vi "CreateClass.vi"(0 "ClassWriterNative":refnum<class "ClassWriterNative.lvclass">, 1 "ProjectTreePosition(String or Project Item Ref)":variant, 2 "CreateClassData":T1, 5 "error in (no error)":errorcluster, 6 "KeepLvClassRefOpen(False)":bool, 7 "HeaderToApply (take from VIRef or /use 2D-8bit header, Ignored if not wired)":variant) -> (14 "ClassWriterNative":refnum<class "ClassWriterNative.lvclass">, 15 "LVClassLibraryRefnum":refnum<vi>, 16 "TemplateVersionUsed":string, 19 "error out":errorcluster)   [LabVIEW 2020, in "ClassWriterNative.lvclass"]
uses:
  <resource>/Framework/Providers/Open_GDS/ClassProviders/Provider_LvNativeClass/ClassWriterNative_class/ClassWriterNative.lvclass
  <resource>/Framework/Providers/Open_GDS/ClassProviders/Provider_BaseClassInterface/CreateClassData.ctl
  <resource>/Framework/Providers/Open_GDS/ClassProviders/Provider_LvNativeClass/LvNativeProviderName.ctl
  <resource>/Framework/Providers/Open_GDS/ClassProviders/Provider_LvNativeClass/Templates/LvNativeTemplateNames.ctl
  <vilib>/Utility/miscctls.llb/LVPositionTypeDef.ctl
  <resource>/Framework/Providers/Open_GDS/ClassProviders/Common/LvClass_class/GDSLvCLass_ClassSettingsType.ctl
  <resource>/Framework/Providers/Open_GDS/ClassProviders/Common/LvClass_class/GDSLvClass_PlugIn.ctl
  <resource>/Framework/Providers/Open_GDS/ClassProviders/Common/LvClass_class/GDSLvClass_PlugInTypes.ctl
  <resource>/Framework/Providers/Open_GDS/ClassProviders/Provider_LvNativeClass/ClassWriterNative_class/ClassWriterNative.lvclass/ClassWriterNative.ctl
  <resource>/Framework/Providers/Open_GDS/ClassProviders/Provider_BaseClassInterface/ClassWriter_class/ClassWriter.lvclass
  <vilib>/Utility/lvfile.llb/NI_FileType.lvlib
  <resource>/Framework/Providers/Open_GDS/ClassProviders/Common/InterfaceLibrary/InterfaceLibrary.lvlib
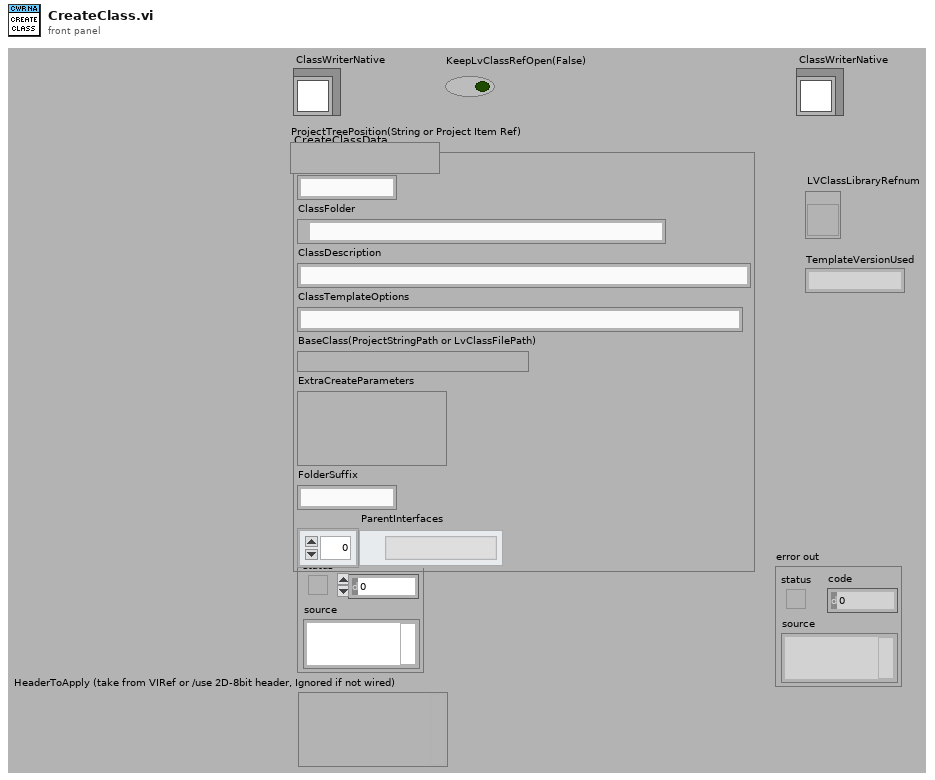
[diagram p1: front panel]
types:
  T1 = typedef "ClassWriter.lvclass/CreateClassData.ctl" = cluster{"ClassName":string, "ClassFolder":path, "ClassDescription":string, "ClassTemplateOptions":string, "BaseClass(ProjectStringPath or LvClassFilePath)":variant, "ExtraCreateParameters":variant, "FolderSuffix":string, "ParentInterfaces":path[]}
  T2 = cluster{"SubClass":bool, "ClassTemplateFiles":path[], "ClassName":string, "ClassFolder":path, "VIs":refnum<vi>[], "TemplateFolder":path, "ViSubDirs":string[], "TemplateName":string, "BaseClassFolder":path, "RootBaseClassFolder":path, "TemplateClass":refnum<vi>, "LvClassPath":path, "ClassRefnum":refnum<vi>, "ProjectRefnum":refnum<vi>, "LvClassFolderPath":path, "BaseClassName":string, "TemplateVersionUsed":string, "App":refnum<vi>}
  T3 = typedef "LvNativeProviderName.ctl" = enum16{"Endevo LabVIEW Native"}
  T4 = enum32{"invalid scope", "public", "private", "protected"}
  T5 = typedef "LVPositionTypeDef.ctl" = cluster{"Left":i32, "Top":i32}
  T6 = typedef "LvNativeTemplateNames.ctl" = enum16{"NativeBaseTemplate", "NativeSubTemplate", "NativeBaseTemplate_4x4x4", "NativeSubTemplate_4x4x4"}
  T7 = typedef "GDSLvCLass_ClassSettingsType.ctl" = cluster{"ClassProviderName":string, "ClassTemplateUsed":string, "ClassTemplateVersion":string, "ClassDescription":string, "PlugIns":T8[], "ConnectorPanePattern":string}
  T8 = typedef "GDSLvClass_PlugIn.ctl" = cluster{"Type":T9, "ID":string, "Version":string, "Path":path, "Name":string, "Data":variant}
  T9 = typedef "GDSLvClass_PlugInTypes.ctl" = enum16{"DesignPattern", "MethodTypes"}
  T10 = typedef "ClassWriter.lvclass/TemplateSettings.ctl" = cluster{"CommonClassTemplate":bool, "DynamicDispatch":enum8{"False", "True", "Mixed"}, "MustOverride":enum8{"False", "True", "Mixed"}, "MustCallParent":enum8{"False", "True", "Mixed"}, "OnlyNormalMethod":bool, "OnlyPublic":bool}
  T11 = cluster{"Major":u16, "Minor":u16, "Fix":u16, "Build":u16}
  T12 = typedef "Scripting_ConnectorPanePatternType.ctl" = u16
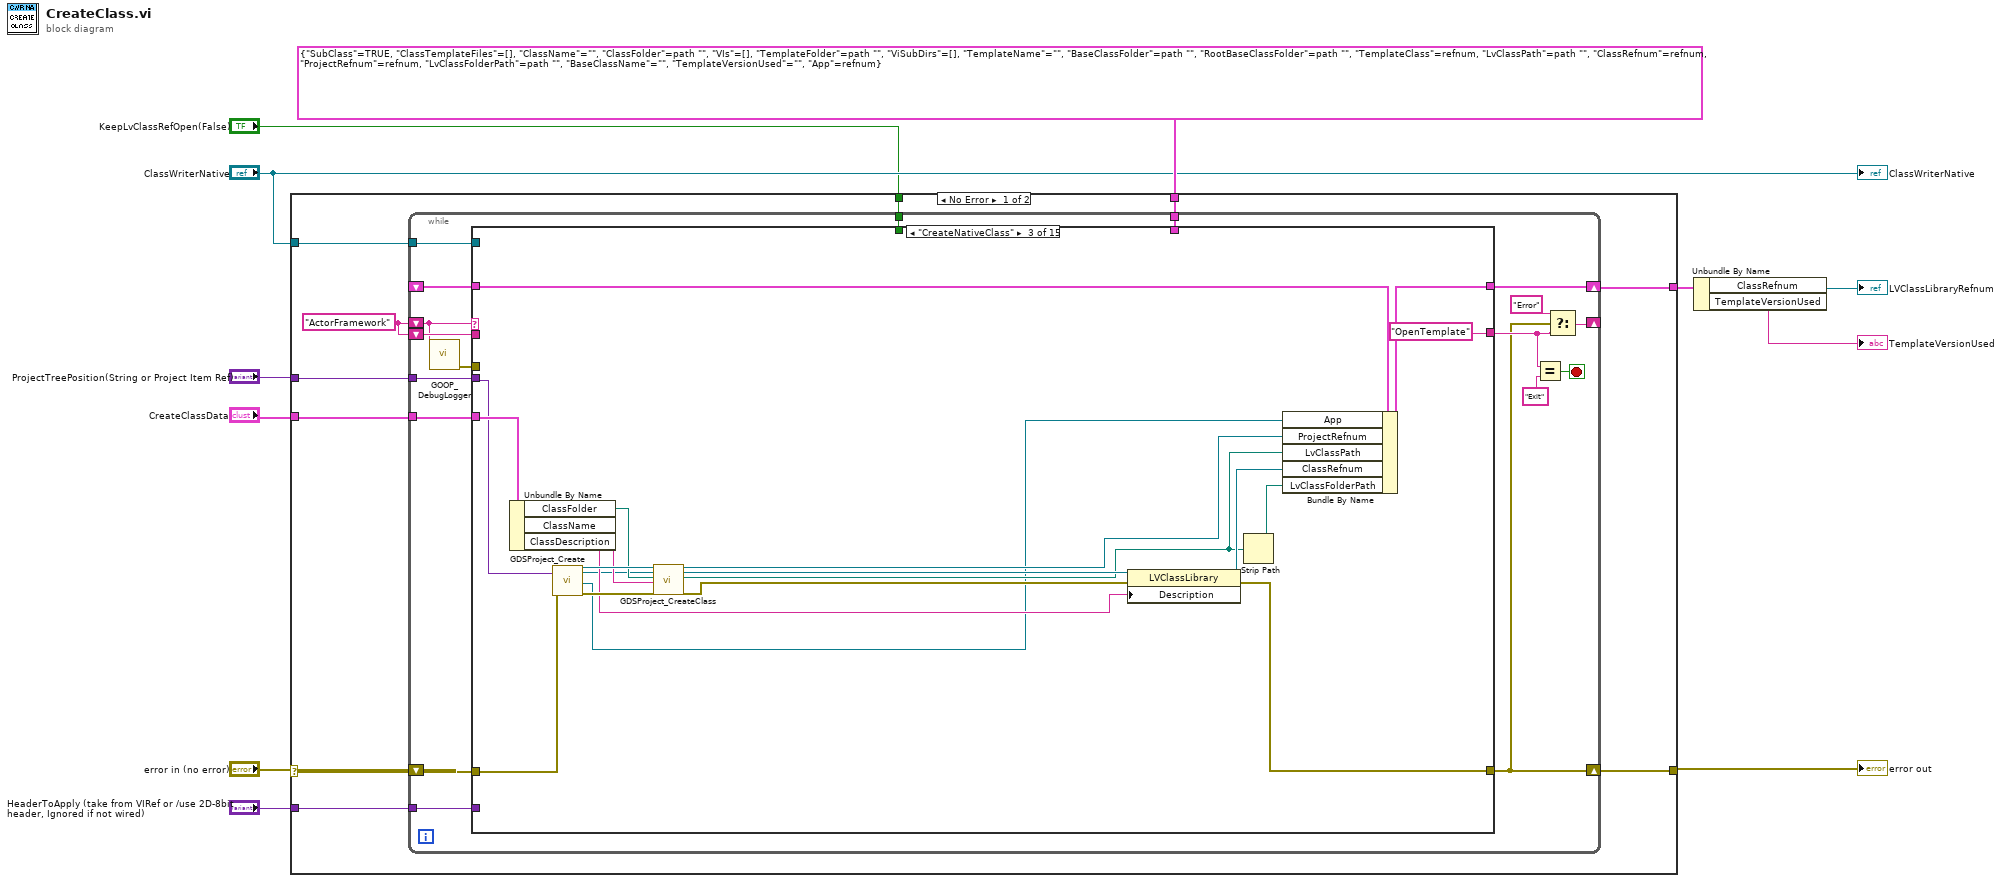
[diagram p0: block diagram]
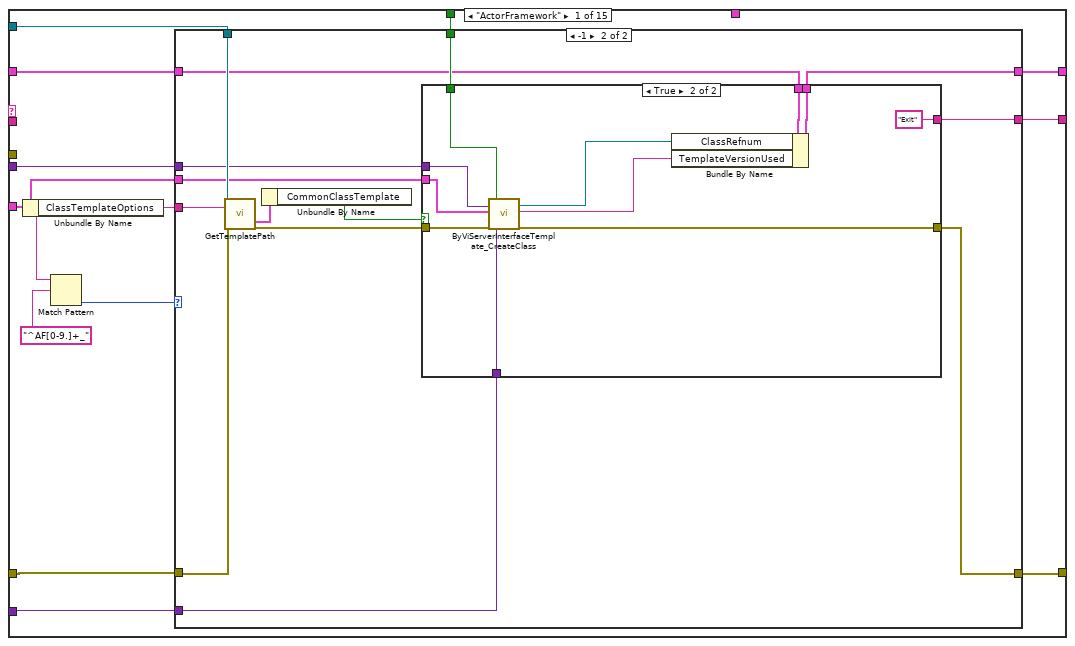
[diagram p2: hidden frame]
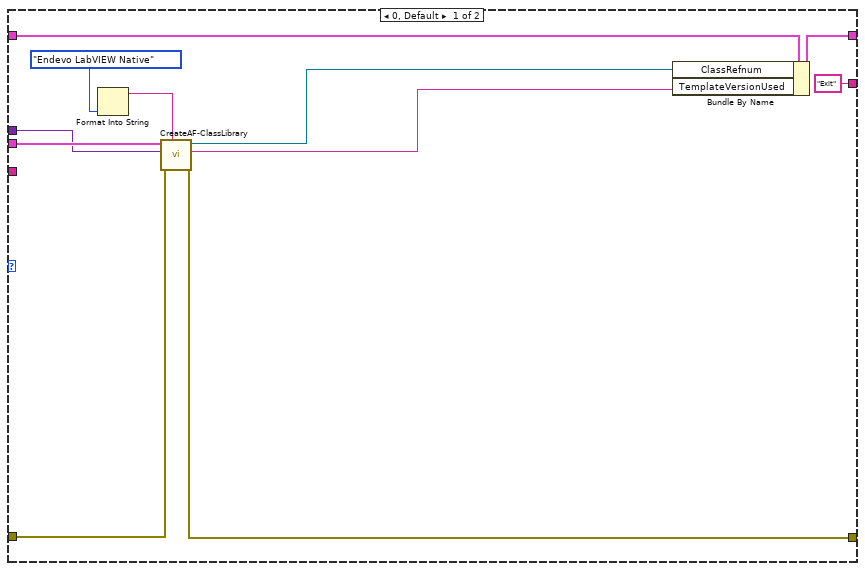
[diagram p3: hidden frame]
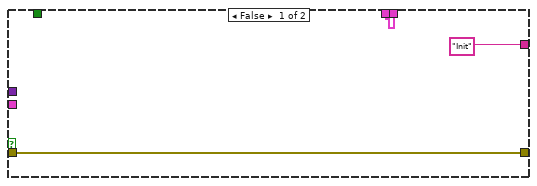
[diagram p4: hidden frame]
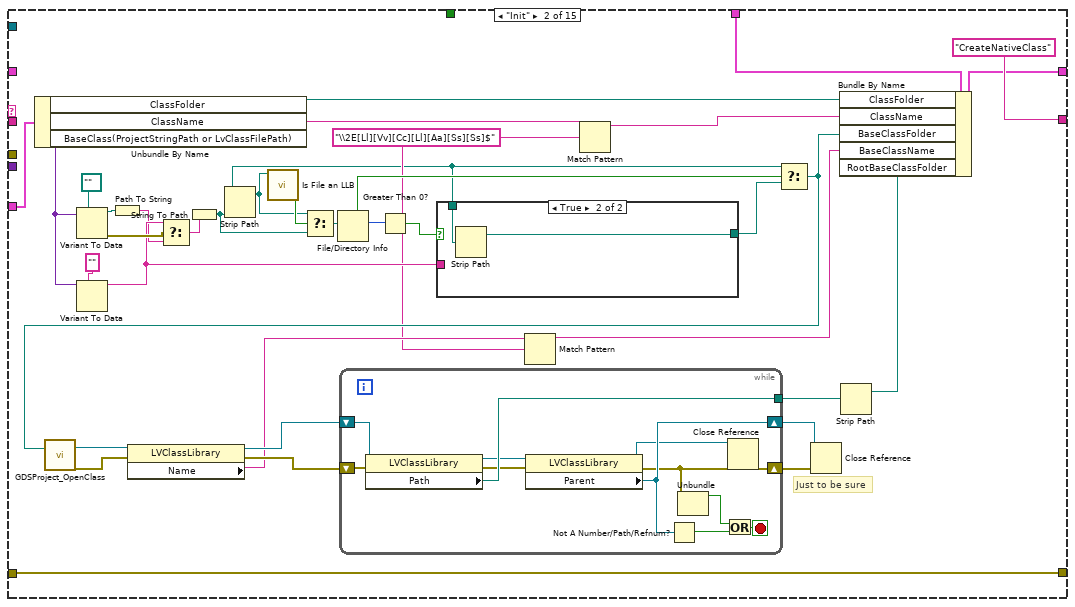
[diagram p5: hidden frame]
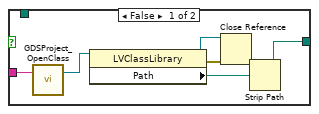
[diagram p6: hidden frame]
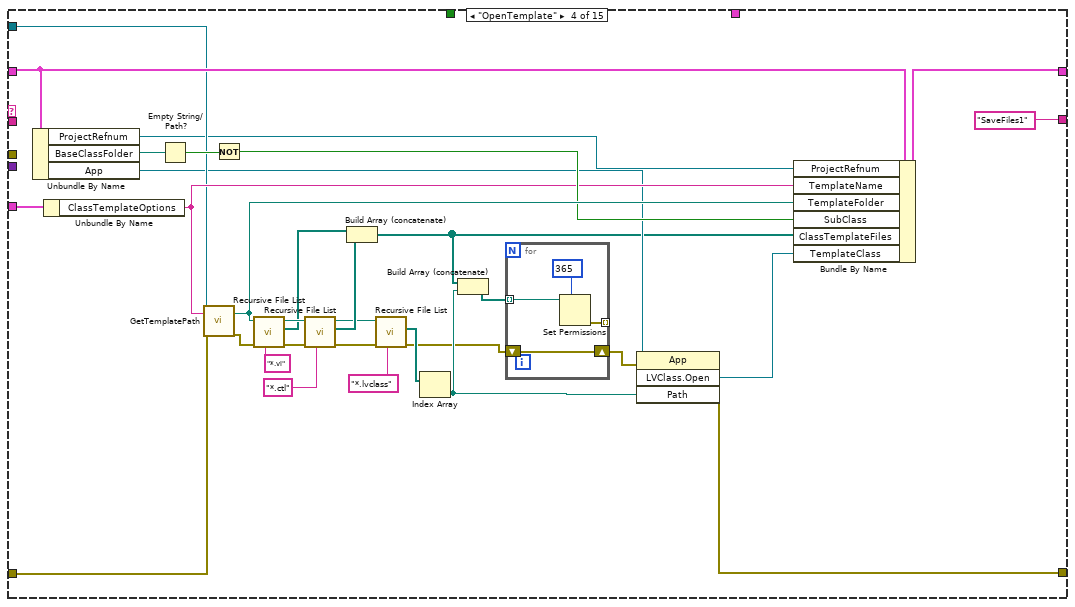
[diagram p7: hidden frame]
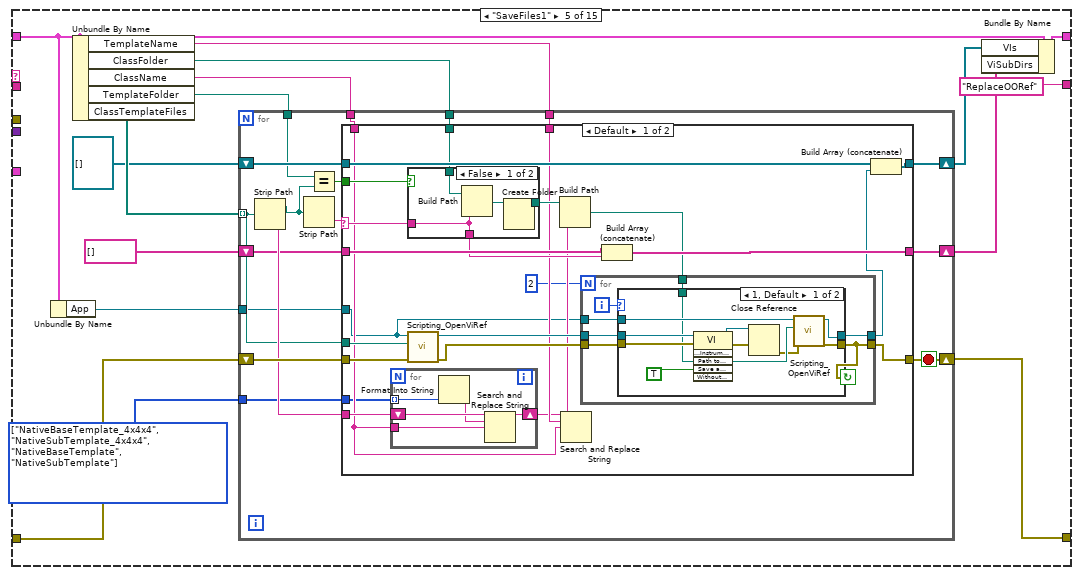
[diagram p8: hidden frame]
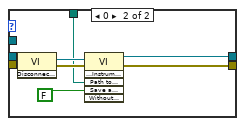
[diagram p9: hidden frame]
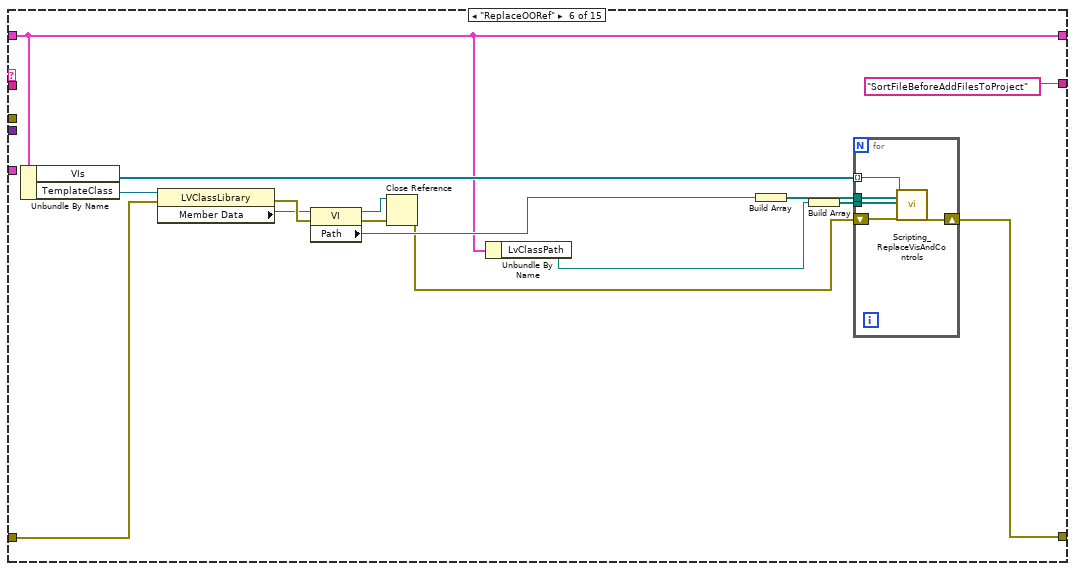
[diagram p12: hidden frame]
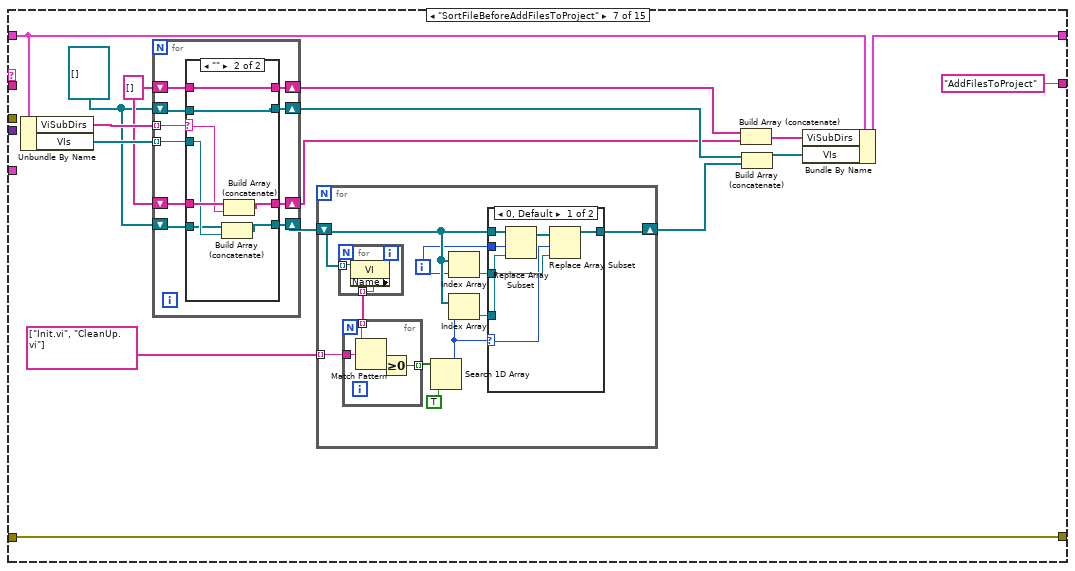
[diagram p13: hidden frame]
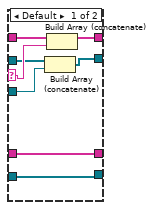
[diagram p15: hidden frame]
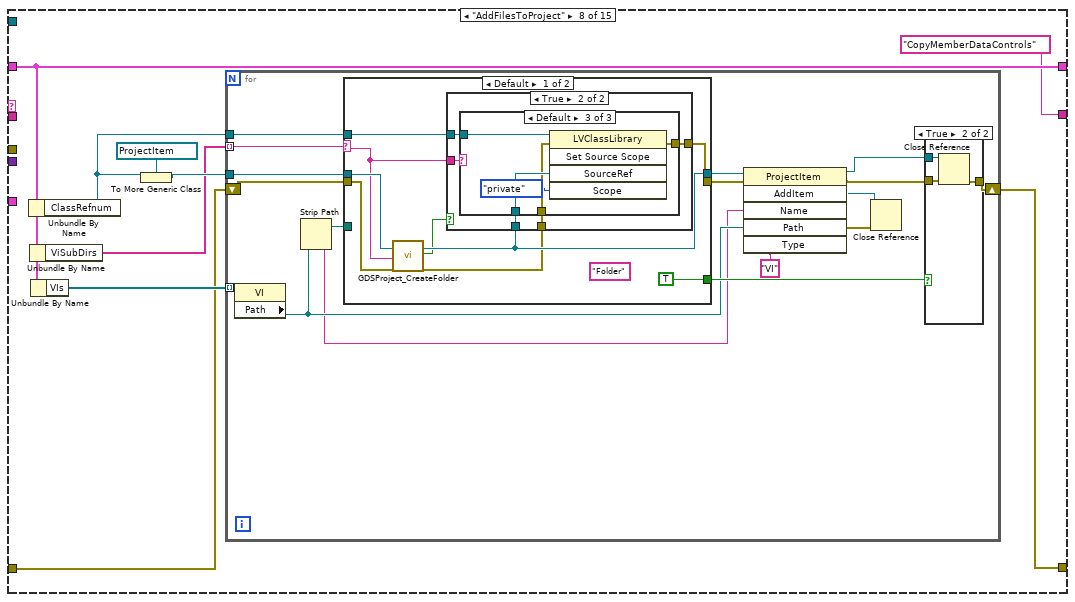
[diagram p16: hidden frame]
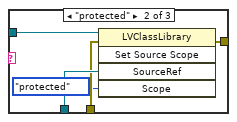
[diagram p20: hidden frame]
diagram:
  n1 = case shown="No Error" "error in (no error)" {
    selector: "error in (no error)" -> [w21 w687]
    tunnel: [w20 w687] -> w7
    tunnel: T2 {"SubClass"=TRUE, "ClassTemplateFiles"=[], "ClassName"="", "ClassFolder"=path "", "VIs"=[], "TemplateFolder"=path "", "ViSubDirs"=[], "TemplateName"="", "BaseClassFolder"=path "", "RootBaseClassFolder"=path "", "TemplateClass"=refnum, "LvClassPath"=path "", "ClassRefnum"=refnum, "ProjectRefnum"=refnum, "LvClassFolderPath"=path "", "BaseClassName"="", "TemplateVersionUsed"="", "App"=refnum} ("output cluster") -> [w19 _]
    tunnel: "ProjectTreePosition(String or Project Item Ref)" -> [w18 _]
    tunnel: "CreateClassData" -> [w17 _]
    tunnel: "ClassWriterNative" -> [w16 _]
    tunnel: "HeaderToApply (take from VIRef or /use 2D-8bit header, Ignored if not wired)" -> [w15 _]
    tunnel: "KeepLvClassRefOpen(False)" -> [w14 _]
    tunnel: [w13 _] -> w3
    frame No Error {
      w12 = "ActorFramework"
      n2 = while {
        shift-right: [w30] -> w20
        shift-left: w21 -> [w39]
        shift-right: [w34] -> _
        shift-left: w12 -> [w23]
        shift-right: [w37] -> w13
        shift-left: _ -> [w38]
        tunnel: w19 -> [w32]
        tunnel: w18 -> [w29]
        tunnel: w17 -> [w28]
        tunnel: w16 -> [w27]
        shift-left: w12 -> [w26]
        tunnel: w15 -> [w25]
        tunnel: w14 -> [w24]
        stop <- w35 stop-if-true
        n3 = call <resource>:"GOOP_DebugLogger.vi"("State"=w23) -> ("error out"=w22:errorcluster)  [unwired: 8 in, 2 out]
        n4 = case shown="\"CreateNativeClass\"" w23 {
          selector: w23 -> [_ _ _ _ _ _ _ _ _ _ _ _ _ _ w662]
          tunnel: w38 -> [w50 _ w154 w183 w206 w299 w331 w386 w491 w506 w525 w546 w560 w637 w659]
          tunnel: [w47 w124 w153 w197 w212 w299 w330 w386 w491 w506 w525 w546 w559 w637 w659] -> w37
          tunnel: w39 -> [w48 w127 w156 w177 w203 w305 w329 w384 w451 w497 w518 w544 w566 w615 w668]
          tunnel: [w45 w127 w152 w172 w202 w310 w329 w391 w441 w494 w529 w538 w583 w616 w661] -> w30
          tunnel: [w46 "CreateNativeClass" "OpenTemplate" "SaveFiles1" "ReplaceOORef" "SortFileBeforeAddFilesToProject" "AddFilesToProject" "CopyMemberDataControls" "UpdateIcons" w508 "AddFolders" "SetClassProperties" "FixAttribute" "CloseRefs" "Exit"] -> w31
          tunnel: w32 -> [_ w112 _ _ _ _ _ _ _ _ _ _ _ _ _]
          tunnel: w29 -> [w44 _ w155 _ _ _ _ _ _ _ _ _ _ _ _]
          tunnel: w28 -> [w49 w111 w157 w179 _ _ _ _ _ _ _ _ w580 _ _]
          tunnel: w27 -> [w42 _ _ w180 _ _ _ _ _ w493 w520 _ _ _ _]
          tunnel: w26 -> [_ _ _ _ _ _ _ _ _ _ _ _ _ _ w660]
          tunnel: w25 -> [w40 _ _ _ _ _ _ _ _ w502 _ _ _ _ _]
          tunnel: w24 -> [w41 _ _ _ _ _ _ _ _ _ _ _ _ _ w657]
          tunnel: w22 -> [_ _ _ _ _ _ _ _ _ _ _ _ _ _ _]
          frame "ActorFramework" {
            n5 = Unbundle By Name(w49) -> ("ClassTemplateOptions"=w43:string)
            n6 = Match Pattern(string=w43, regular expression="^AF[0-9.]+_") -> (offset past match=w52:i32)  [unwired: 1 in, 3 out]
            n7 = case shown="-1" w52 {
              tunnel: w50 -> [w63 w67]
              tunnel: [w62 w66] -> w47
              tunnel: ["Exit" w74] -> w46
              tunnel: w49 -> [w60 w69]
              tunnel: w48 -> [w59 w75]
              tunnel: [w58 w72] -> w45
              tunnel: w44 -> [w53 w70]
              tunnel: w43 -> [_ w77]
              tunnel: w42 -> [_ w76]
              tunnel: w41 -> [_ w71]
              tunnel: w40 -> [_ w68]
              frame 0, Default {
                n8 = Format Into String(LvNativeProviderName."Endevo LabVIEW Native" ("ProviderName")) -> (resulting string=w57:string)  [unwired: 3 in, 1 out]
                n9 = call <resource>:"CreateAF-ClassLibrary.vi"("Providername"=w57, "error in (no error)"=w59, "ProjectTreePosition(String or Project Item Ref)"=w53, "CreateClassData"=w60) -> ("error out"=w58:errorcluster, "TemplateVersionUsed"=w55:string, "LVClassLibraryRefnum"=w56:refnum<vi>)  [unwired: 5 in]
                n10 = Bundle By Name(cluster=w63, "ClassRefnum"=w56, "TemplateVersionUsed"=w55) -> (w62:T2)
              }
              frame -1 {
                n11 = call-dynamic "GetTemplatePath.vi"("reference in"=w76, "ClassTemplateSubDirectory"=w77, "error in (no error)"=w75) -> ("TemplateSettings"=w65:T10, "error out"=w73:errorcluster)  [unwired: 12 in, 3 out]
                n12 = Unbundle By Name(w65) -> ("CommonClassTemplate"=w64:bool)
                n13 = case shown="True" w64 {
                  tunnel: ["Init" "Exit"] -> w74
                  tunnel: w73 -> [w79 w90]
                  tunnel: [w79 w89] -> w72
                  tunnel: w71 -> [_ w88]
                  tunnel: w70 -> [_ w87]
                  tunnel: w69 -> [_ w86]
                  tunnel: w68 -> [_ w85]
                  tunnel: w67 -> [w78 w84]
                  tunnel: [w78 w83] -> w66
                  frame False {
                  }
                  frame True {
                    n14 = call <resource>:"ByViServerInterfaceTemplate_CreateClass.vi"("ProjectTreePosition(String or Project Item Ref)"=w87, "CreateClassData"=w86, "error in (no error)"=w90, "KeepLvClassRefOpen(False)"=w88, "HeaderToApply (take from VIRef or /use 2D-8bit header, Ignored if not wired)"=w85) -> ("LVClassLibraryRefnum"=w82:refnum<vi>, "TemplateVersionUsed"=w81:string, "error out"=w89:errorcluster)  [unwired: 12 in]
                    n15 = Bundle By Name(cluster=w84, "ClassRefnum"=w82, "TemplateVersionUsed"=w81) -> (w83:T2)
                  }
                }
              }
            }
          }
          frame "Init" {
            w97 = "\\2E[Ll][Vv][Cc][Ll][Aa][Ss][Ss]$" ("regular expression")
            # "Just to be sure"
            n16 = Unbundle By Name(w111) -> ("ClassFolder"=w110:path, "ClassName"=w109:string, "BaseClass(ProjectStringPath or LvClassFilePath)"=w108:variant)
            n17 = Variant To Data(type=path "" ("path"), Variant=w108) -> (data=w114:path, error out=w118:errorcluster)  [unwired: 1 in]
            n18 = Variant To Data(type="" ("regular expression"), Variant=w108) -> (data=w115:string)  [unwired: 1 in, 1 out]
            n19 = Path To String(path=w114) -> (string=w113:string)
            n20 = Select(t=w115, s=w118, f=w113) -> (s? t:f=w117:string)
            n21 = String To Path(string=w117) -> (path=w93:path)
            n22 = Strip Path(path=w93) -> (stripped path=w94:path)  [unwired: 1 out]
            n23 = call <vilib>:"Is File an LLB.vi"("path"=w94) -> ("Is LLB?"=w95:bool)  [unwired: 9 in, 1 out]
            n24 = Select(t=w94, s=w95, f=w93) -> (s? t:f=w92:path)
            n25 = File/Directory Info(path=w92) -> (directory=w122:bool, size=w121:i64)  [unwired: 1 in, 5 out]
            n26 = Greater Than 0?(x=w121) -> (x > 0?=w119:bool)
            n27 = case shown="True" w119 {
              tunnel: w93 -> [_ w146]
              tunnel: [w143 w145] -> w120
              tunnel: w115 -> [w144 _]
              frame False {
                n28 = call <resource>:"GDSProject_OpenClass.vi"("ClassPath(FilePath/ProjectTreePath/LvCLassRef)"=w144) -> ("LVClass.Open"=w141:refnum<vi>)  [unwired: 16 in, 2 out]
                n29 = property class="LVClassLibrary"(reference=w141) -> (reference out=w139:refnum<vi>, error out=w140:errorcluster, "Path"=w142:path)  [unwired: 1 in]
                n30 = Close Reference(reference=w139, error in (no error)=w140) -> ()  [unwired: 1 out]
                n31 = Strip Path(path=w142) -> (stripped path=w143:path)  [unwired: 1 out]
              }
              frame True {
                n32 = Strip Path(path=w146) -> (stripped path=w145:path)  [unwired: 1 out]
              }
            }
            n33 = Match Pattern(string=w109, regular expression=w97) -> (before substring=w125:string)  [unwired: 1 in, 3 out]
            n34 = Select(t=w93, s=w122, f=w120) -> (s? t:f=w107:path)
            n35 = call <resource>:"GDSProject_OpenClass.vi"("ClassPath(FilePath/ProjectTreePath/LvCLassRef)"=w107) -> ("LVClass.Open"=w100:refnum<vi>, "error out"=w102:errorcluster)  [unwired: 16 in, 1 out]
            n36 = property class="LVClassLibrary"(reference=w100, error in=w102) -> (reference out=w99:refnum<vi>, error out=w101:errorcluster, "Name"=w98:string)
            n37 = while {
              shift-right: [w135] -> w106
              shift-left: w101 -> [w130]
              shift-right: [w136] -> w105
              shift-left: w99 -> [w138]
              tunnel: [w137] -> w104
              stop <- w132 stop-if-true
              n38 = property class="LVClassLibrary"(reference=w138, error in=w130) -> (reference out=w128:refnum<vi>, error out=w129:errorcluster, "Path"=w137:path)
              n39 = property class="LVClassLibrary"(reference=w128, error in=w129) -> (reference out=w131:refnum<vi>, error out=w135:errorcluster, "Parent"=w136:refnum<vi>)
              n40 = Not A Number/Path/Refnum?(number/path/refnum=w136) -> (NaN/Path/Refnum?=w133:bool)
              n41 = Unbundle(w135) -> ("status"=w134:bool)  [unwired: 2 out]
              n42 = Or(x=w134, y=w133) -> (x .or. y?=w132:bool)
              n43 = Close Reference(reference=w131) -> ()  [unwired: 1 in, 1 out]
            }
            n44 = Match Pattern(string=w98, regular expression=w97) -> (before substring=w96:string)  [unwired: 1 in, 3 out]
            n45 = Close Reference(reference=w105, error in (no error)=w106) -> ()  [unwired: 1 out]
            n46 = Strip Path(path=w104) -> (stripped path=w103:path)  [unwired: 1 out]
            n47 = Bundle By Name(cluster=w112, "ClassFolder"=w110, "ClassName"=w125, "BaseClassFolder"=w107, "BaseClassName"=w96, "RootBaseClassFolder"=w103) -> (w124:T2)
          }
          frame "CreateNativeClass" {
            n48 = Unbundle By Name(w157) -> ("ClassFolder"=w161:path, "ClassName"=w162:string, "ClassDescription"=w158:string)
            n49 = call <resource>:"GDSProject_Create.vi"("ProjectTreePosition(String or Project Item Ref)"=w155, "error in (no error)"=w156) -> ("Project Refnum"=w165:refnum<vi>, "Project Item"=w151:refnum<vi>, "App"=w147:refnum<vi>, "error out"=w164:errorcluster)  [unwired: 13 in, 1 out]
            n50 = call <resource>:"GDSProject_CreateClass.vi"("Project Refnum In"=w165, "Project Item To Create Class Below(Use MyComputer if not wired)"=w151, "ClassFolder"=w161, "ClassName"=w162, "error in (no error)"=w164) -> ("Project Refnum Out"=w149:refnum<vi>, "Class Refnum Out"=w160:refnum<vi>, "ClassPathOut"=w150:path, "error out"=w148:errorcluster)  [unwired: 11 in]
            n51 = property class="LVClassLibrary"(reference=w160, error in=w148, "Description"=w158) -> (reference out=w159:refnum<vi>, error out=w152:errorcluster)
            n52 = Strip Path(path=w150) -> (stripped path=w163:path)  [unwired: 1 out]
            n53 = Bundle By Name(cluster=w154, "App"=w147, "ProjectRefnum"=w149, "LvClassPath"=w150, "ClassRefnum"=w159, "LvClassFolderPath"=w163) -> (w153:T2)
          }
          frame "OpenTemplate" {
            n54 = Unbundle By Name(w183) -> ("ProjectRefnum"=w174:refnum<vi>, "BaseClassFolder"=w185:path, "App"=w173:refnum<vi>)
            n55 = Unbundle By Name(w179) -> ("ClassTemplateOptions"=w181:string)
            n56 = Empty String/Path?(string/path=w185) -> (empty?=w184:bool)
            n57 = call-dynamic "GetTemplatePath.vi"("reference in"=w180, "ClassTemplateSubDirectory"=w181, "error in (no error)"=w177) -> ("FolderPathOut"=w186:path, "error out"=w176:errorcluster)  [unwired: 12 in, 3 out]
            n58 = Not(x=w184) -> (.not. x?=w182:bool)
            n59 = call <vilib>:"Recursive File List.vi"("pattern"="*.vi", "error in (no error)"=w176, "Folder Path"=w186) -> ("error out"=w191:errorcluster, "All Files in Dir"=w193:path[], "dup Folder Path"=w195:path)  [unwired: 4 in, 2 out]
            n60 = call <vilib>:"Recursive File List.vi"("pattern"="*.ctl", "error in (no error)"=w191, "Folder Path"=w195) -> ("error out"=w190:errorcluster, "All Files in Dir"=w192:path[], "dup Folder Path"=w189:path)  [unwired: 4 in, 2 out]
            n61 = Build Array (concatenate)(w193, w192) -> (w171:path[])
            n62 = call <vilib>:"Recursive File List.vi"("pattern"="*.lvclass", "error in (no error)"=w190, "Folder Path"=w189) -> ("error out"=w169:errorcluster, "All Files in Dir"=w187:path[])  [unwired: 4 in, 3 out]
            n63 = Index Array(array=w187) -> (element=w170:path)  [unwired: 1 in]
            n64 = Build Array (concatenate)(w171, w170) -> (w167:path[])
            n65 = for {
              tunnel: w167 -> [w200] mode=indexing
              shift-right: [w201] -> w168
              shift-left: w169 -> [w201]
              tunnel: [w198] -> _ mode=indexing
              n66 = Set Permissions(7:i16 365 ("permissions"), 11:w200) -> (0:w198:errorcluster)  [unwired: 3 in, 1 out]
            }
            n67 = invoke class="App" method="LVClass.Open"(reference=w173, error in=w168, "Path"=w170) -> (error out=w172:errorcluster, "LVClass.Open"=w175:refnum<vi>)  [unwired: 1 in, 2 out]
            n68 = Bundle By Name(cluster=w183, "ProjectRefnum"=w174, "TemplateName"=w181, "TemplateFolder"=w186, "SubClass"=w182, "ClassTemplateFiles"=w171, "TemplateClass"=w175) -> (w197:T2)
          }
          frame "SaveFiles1" {
            w205 = T6[] [enum."NativeBaseTemplate_4x4x4", enum."NativeSubTemplate_4x4x4", enum."NativeBaseTemplate", enum."NativeSubTemplate"] items=["NativeBaseTemplate", "NativeSubTemplate", "NativeBaseTemplate_4x4x4", "NativeSubTemplate_4x4x4"]
            n69 = Unbundle By Name(w206) -> ("App"=w204:refnum<vi>)
            n70 = Unbundle By Name(w206) -> ("TemplateName"=w207:string, "ClassFolder"=w216:path, "ClassName"=w215:string, "TemplateFolder"=w210:path, "ClassTemplateFiles"=w217:path[])
            n71 = for {
              tunnel: w217 -> [w223] mode=indexing
              shift-right: [w228] -> w213
              shift-left: refnum<vi>[] [] -> [w229]
              shift-right: [w218] -> w202
              shift-left: w203 -> [w233]
              tunnel: w216 -> [w232]
              tunnel: w215 -> [w230]
              tunnel: w210 -> [w225]
              shift-right: [w224] -> w208
              shift-left: string[] [] -> [w222]
              tunnel: w204 -> [w221]
              tunnel: w207 -> [w220]
              tunnel: w205 -> [w219]
              stop <- w218 stop-if-true
              n72 = Strip Path(path=w223) -> (stripped path=w227:path, name=w231:string)
              n73 = Strip Path(path=w227) -> (name=w234:string)  [unwired: 1 out]
              n74 = Equal?(x=w225, y=w227) -> (x = y?=w226:bool)
              n75 = case shown="Default" w234 {
                selector: w234 -> [w252 _]
                tunnel: w223 -> [w258 _]
                tunnel: w233 -> [w257 w295]
                tunnel: [w244 w295] -> w218
                tunnel: w232 -> [w253 _]
                tunnel: w231 -> [w256 _]
                tunnel: w230 -> [w239 _]
                tunnel: w229 -> [w255 w296]
                tunnel: [w254 w296] -> w228
                tunnel: w226 -> [w250 _]
                tunnel: [w248 w294] -> w224
                tunnel: w222 -> [w249 w294]
                tunnel: w221 -> [w236 _]
                tunnel: w220 -> [w240 _]
                tunnel: w219 -> [w237 _]
                frame Default {
                  n76 = for {
                    tunnel: w239 -> [w286]
                    shift-right: [w288] -> w238
                    shift-left: w256 -> [w287]
                    tunnel: w237 -> [w285] mode=indexing
                    n77 = Format Into String(w285) -> (resulting string=w284:string)  [unwired: 3 in, 1 out]
                    n78 = Search and Replace String(input string=w287, search string=w284, replace string=w286) -> (result string=w288:string)  [unwired: 5 in, 3 out]
                  }
                  n79 = case shown="False" w250 {
                    tunnel: w253 -> [w292 w293]
                    tunnel: w252 -> [w289 _]
                    tunnel: [w290 w293] -> w251
                    tunnel: [w289 _] -> w247
                    frame False {
                      n80 = Build Path(base path=w292, name or relative path=w289) -> (appended path=w291:path)
                      n81 = Create Folder(path (use dialog)=w291) -> (created path=w290:path)  [unwired: 2 in, 2 out]
                    }
                    frame True {
                    }
                  }
                  n82 = call <resource>:"Scripting_OpenViRef.vi"("error in"=w257, "ViPath/ViName/Viref"=w258, "AppRef"=w236) -> ("error out"=w246:errorcluster, "vi reference"=w245:refnum<vi>)  [unwired: 6 in, 1 out]
                  n83 = Search and Replace String(input string=w238, search string=w240, replace string=w239) -> (result string=w241:string)  [unwired: 5 in, 3 out]
                  n84 = Build Path(base path=w251, name or relative path=w241) -> (appended path=w242:path)
                  n85 = for {
                    N: 2 -> [_]
                    tunnel: w242 -> [w262]
                    tunnel: w236 -> [w261]
                    tunnel: w246 -> [w265]
                    tunnel: [w259] -> w244
                    tunnel: w245 -> [w264]
                    tunnel: [w263] -> w243
                    i -> [w260]
                    stop <- w259 continue-if-true
                    n86 = case shown="1, Default" w260 {
                      tunnel: w265 -> [w274 w283]
                      tunnel: w264 -> [w275 w282]
                      tunnel: [w270 w279] -> w259
                      tunnel: [w269 w278] -> w263
                      tunnel: w262 -> [w271 w277]
                      tunnel: w261 -> [w272 _]
                      frame 1, Default {
                        n87 = invoke class="VI" method="Save.Instrument"(reference=w275, error in=w274, "Path to saved file"=w271, "Save a Copy"=TRUE) -> (reference out=w267:refnum<vi>, error out=w268:errorcluster)  [unwired: 2 in, 4 out]
                        n88 = Close Reference(reference=w267, error in (no error)=w268) -> (error out=w266:errorcluster)
                        n89 = call <resource>:"Scripting_OpenViRef.vi"("error in"=w266, "ViPath/ViName/Viref"=w271, "AppRef"=w272) -> ("error out"=w270:errorcluster, "vi reference"=w269:refnum<vi>)  [unwired: 6 in, 1 out]
                      }
                      frame 0 {
                        n90 = invoke class="VI" method="DisconnectFromLibrary"(reference=w282, error in=w283) -> (reference out=w281:refnum<vi>, error out=w280:errorcluster)  [unwired: 1 in, 1 out]
                        n91 = invoke class="VI" method="Save.Instrument"(reference=w281, error in=w280, "Path to saved file"=w277, "Save a Copy"=FALSE) -> (reference out=w278:refnum<vi>, error out=w279:errorcluster)  [unwired: 2 in, 4 out]
                      }
                    }
                  }
                  n92 = Build Array (concatenate)(w249, w247) -> (w248:string[])
                  n93 = Build Array (concatenate)(w255, w243) -> (w254:refnum<vi>[])
                }
                frame "methods" {
                }
              }
            }
            n94 = Bundle By Name(cluster=w206, "VIs"=w213, "ViSubDirs"=w208) -> (w212:T2)
          }
          frame "ReplaceOORef" {
            n95 = Unbundle By Name(w299) -> ("VIs"=w311:refnum<vi>[], "TemplateClass"=w306:refnum<vi>)
            n96 = property class="LVClassLibrary"(reference=w306, error in=w305) -> (error out=w308:errorcluster, "Member Data"=w307:refnum<vi>)  [unwired: 1 out]
            n97 = property class="VI"(reference=w307, error in=w308) -> (reference out=w300:refnum<vi>, error out=w301:errorcluster, "Path"=w304:path)
            n98 = Close Reference(reference=w300, error in (no error)=w301) -> (error out=w297:errorcluster)
            n99 = Unbundle By Name(w299) -> ("LvClassPath"=w298:path)
            n100 = Build Array(w304) -> (w303:path[])
            n101 = Build Array(w298) -> (w302:path[])
            n102 = for {
              tunnel: w311 -> [w314] mode=indexing
              shift-right: [w315] -> w310
              shift-left: w297 -> [w316]
              tunnel: w302 -> [w313]
              tunnel: w303 -> [w312]
              n103 = call <resource>:"Scripting_ReplaceVisAndControls.vi"("ViRef"=w314, "OldVIsAndControls"=w312, "NewVIsAndControls"=w313, "error in (no error)"=w316) -> ("error out"=w315:errorcluster)  [unwired: 14 in, 1 out]
            }
          }
          frame "SortFileBeforeAddFilesToProject" {
            w321 = refnum<vi>[] []
            w322 = string[] []
            n104 = Unbundle By Name(w331) -> ("ViSubDirs"=w328:string[], "VIs"=w327:refnum<vi>[])
            n105 = for {
              tunnel: w328 -> [w366] mode=indexing
              tunnel: w327 -> [w361] mode=indexing
              shift-right: [w364] -> w326
              shift-left: w322 -> [w365]
              shift-right: [w362] -> w323
              shift-left: w321 -> [w363]
              shift-right: [w358] -> w320
              shift-left: w322 -> [w357]
              shift-right: [w360] -> w319
              shift-left: w321 -> [w359]
              n106 = case shown="\"\"" w366 {
                selector: w366 -> [w372 w378]
                tunnel: w365 -> [w374 w382]
                tunnel: [w373 w382] -> w364
                tunnel: w363 -> [w371 w381]
                tunnel: [w370 w381] -> w362
                tunnel: w361 -> [w369 w377]
                tunnel: w357 -> [w368 w380]
                tunnel: [w368 w379] -> w358
                tunnel: w359 -> [w367 w376]
                tunnel: [w367 w375] -> w360
                frame Default {
                  n107 = Build Array (concatenate)(w371, w369) -> (w370:refnum<vi>[])
                  n108 = Build Array (concatenate)(w374, w372) -> (w373:string[])
                }
                frame "" {
                  n109 = Build Array (concatenate)(w376, w377) -> (w375:refnum<vi>[])
                  n110 = Build Array (concatenate)(w380, w378) -> (w379:string[])
                }
              }
            }
            n111 = for {
              shift-right: [w338] -> w317
              shift-left: w319 -> [w342]
              tunnel: string[] ["Init.vi", "CleanUp.vi"] -> [w336] mode=indexing
              i -> [w341]
              n112 = for {
                tunnel: w342 -> [w356] mode=indexing
                tunnel: [w355] -> w337 mode=indexing
                n113 = property class="VI"(reference=w356) -> ("Name"=w355:string)  [unwired: 1 in, 2 out]
              }
              n114 = for {
                tunnel: w337 -> [w346] mode=indexing
                tunnel: w336 -> [w345]
                tunnel: [w343] -> w335 mode=indexing
                n115 = Match Pattern(string=w346, regular expression=w345) -> (offset past match=w344:i32)  [unwired: 1 in, 3 out]
                n116 = Greater Or Equal To 0?(x=w344) -> (x >= 0?=w343:bool)
              }
              n117 = Search 1D Array(1D array=w335, element=TRUE) -> (index of element=w333:i32)  [unwired: 1 in]
              n118 = Index Array(array=w342, index=w341) -> (element=w339:refnum<vi>)
              n119 = Index Array(array=w342, index=w333) -> (element=w340:refnum<vi>)
              n120 = case shown="0, Default" w333 {
                selector: w333 -> [w348 _]
                tunnel: w342 -> [w353 w354]
                tunnel: w341 -> [w352 _]
                tunnel: w340 -> [w351 _]
                tunnel: w339 -> [w349 _]
                tunnel: [w347 w354] -> w338
                frame 0, Default {
                  n121 = Replace Array Subset(array=w353, new element=w351, index=w352) -> (w350:refnum<vi>[])
                  n122 = Replace Array Subset(array=w350, new element=w349, index=w348) -> (w347:refnum<vi>[])
                }
                frame -1 {
                }
              }
            }
            n123 = Build Array (concatenate)(w326, w320) -> (w325:string[])
            n124 = Build Array (concatenate)(w323, w317) -> (w324:refnum<vi>[])
            n125 = Bundle By Name(cluster=w331, "ViSubDirs"=w325, "VIs"=w324) -> (w330:T2)
          }
          frame "AddFilesToProject" {
            n126 = Unbundle By Name(w386) -> ("ClassRefnum"=w385:refnum<vi>)
            n127 = Unbundle By Name(w386) -> ("ViSubDirs"=w388:string[])
            n128 = Unbundle By Name(w386) -> ("VIs"=w387:refnum<vi>[])
            n129 = To More Generic Class(target class=refnum<vi> refnum ("AddItem"), reference=w385) -> (generic class reference=w389:refnum<vi>)
            n130 = for {
              tunnel: w388 -> [w396] mode=indexing
              tunnel: w389 -> [w405]
              shift-right: [w401] -> w391
              shift-left: w384 -> [w403]
              tunnel: w385 -> [w395]
              tunnel: w387 -> [w397] mode=indexing
              n131 = property class="VI"(reference=w397) -> ("Path"=w398:path)  [unwired: 1 in, 2 out]
              n132 = Strip Path(path=w398) -> (stripped path=w406:path, name=w394:string)
              n133 = case shown="Default" w396 {
                selector: w396 -> [w414 _]
                tunnel: w405 -> [w420 w439]
                tunnel: [w417 w439] -> w404
                tunnel: w403 -> [w419 w438]
                tunnel: [w415 w438] -> w407
                tunnel: w406 -> [_ _]
                tunnel: w395 -> [w418 _]
                tunnel: [TRUE _] -> w399
                frame Default {
                  (unwired) "Folder"
                  n134 = call <resource>:"GDSProject_CreateFolder.vi"("Project Item To Create Folder Below(Use MyComputer if not wired)"=w420, "FolderName"=w414, "error in (no error)"=w419) -> ("ItemOut"=w417:refnum<vi>, "FolderCreated"=w412:bool, "error out"=w416:errorcluster)  [unwired: 13 in, 1 out]
                  n135 = case shown="True" w412 {
                    tunnel: w418 -> [_ w426]
                    tunnel: w417 -> [_ w425]
                    tunnel: w416 -> [w421 w424]
                    tunnel: [w421 w423] -> w415
                    tunnel: w414 -> [_ w422]
                    frame False {
                    }
                    frame True {
                      n136 = case shown="Default" w422 {
                        tunnel: w426 -> [_ w432 w437]
                        tunnel: w425 -> [_ w431 w436]
                        tunnel: w424 -> [w427 w430 w435]
                        tunnel: [w427 w429 w434] -> w423
                        frame "Public", "util", "utils" {
                        }
                        frame "protected" {
                          n137 = invoke class="LVClassLibrary" method="Set Source Scope"(reference=w432, error in=w430, "SourceRef"=w431, "Scope"=T4."protected" ("scope")) -> (error out=w429:errorcluster)  [unwired: 1 in, 4 out]
                        }
                        frame Default {
                          n138 = invoke class="LVClassLibrary" method="Set Source Scope"(reference=w437, error in=w435, "SourceRef"=w436, "Scope"=T4."private" ("scope")) -> (error out=w434:errorcluster)  [unwired: 1 in, 4 out]
                        }
                      }
                    }
                  }
                }
                frame "" {
                }
              }
              n139 = invoke class="ProjectItem" method="AddItem"(reference=w404, error in=w407, "Name"=w394, "Path"=w398, "Type"="VI") -> (reference out=w400:refnum<vi>, error out=w393:errorcluster, "AddItem"=w392:refnum<vi>)  [unwired: 1 in, 3 out]
              n140 = Close Reference(reference=w392, error in (no error)=w393) -> ()  [unwired: 1 out]
              n141 = case shown="True" w399 {
                tunnel: w393 -> [w408 w411]
                tunnel: [w408 w410] -> w401
                tunnel: w400 -> [_ w409]
                frame False {
                }
                frame True {
                  n142 = Close Reference(reference=w409, error in (no error)=w411) -> (error out=w410:errorcluster)
                }
              }
            }
          }
          frame "CopyMemberDataControls" {
            n143 = Unbundle By Name(w491) -> ("TemplateClass"=w449:refnum<vi>, "ClassRefnum"=w442:refnum<vi>)
            n144 = invoke class="App" method="Clipboard.Empty"(error in=w451) -> (error out=w450:errorcluster)  [unwired: 2 in, 2 out]
            n145 = property class="LVClassLibrary"(reference=w449, error in=w450) -> (error out=w490:errorcluster, "Member Data"=w489:refnum<vi>)  [unwired: 1 out]
            n146 = property class="VI"(reference=w489, error in=w490, "Front Panel.Open"=FALSE ("Front Panel Window:Open")) -> (reference out=w448:refnum<vi>, error out=w486:errorcluster, "Panel"=w487:refnum<vi>)
            n147 = property class="Pnl"(reference=w487, error in=w486) -> (reference out=w483:refnum<vi>, error out=w480:errorcluster, "Controls[]"=w488:refnum<vi>[])
            n148 = Index Array(array=w488) -> (element=w484:refnum<vi>)  [unwired: 1 in]
            n149 = property class="Ctl"(reference=w484, error in=w480, "Selected"=TRUE) -> (reference out=w455:refnum<vi>, error out=w481:errorcluster)
            n150 = invoke class="Pnl" method="Copy Selection"(reference=w483, error in=w481) -> (reference out=w454:refnum<vi>, error out=w472:errorcluster)  [unwired: 1 in, 1 out]
            n151 = property class="LVClassLibrary"(reference=w442, error in=w472) -> (error out=w473:errorcluster, "Member Data"=w474:refnum<vi>)  [unwired: 1 out]
            n152 = property class="VI"(reference=w474, error in=w473, "Front Panel.Open"=FALSE ("Front Panel Window:Open")) -> (reference out=w446:refnum<vi>, error out=w477:errorcluster, "Panel"=w476:refnum<vi>)
            n153 = property class="Pnl"(reference=w476, error in=w477) -> (reference out=w468:refnum<vi>, error out=w479:errorcluster, "Controls[]"=w475:refnum<vi>[])
            n154 = Index Array(array=w475) -> (element=w478:refnum<vi>)  [unwired: 1 in]
            n155 = property class="Ctl"(reference=w478, error in=w479) -> (reference out=w470:refnum<vi>, error out=w471:errorcluster, "Position"=w462:T5)
            n156 = invoke class="Ctl" method="Delete"(reference=w470, error in=w471) -> (reference out=w461:refnum<vi>, error out=w469:errorcluster)  [unwired: 1 in, 1 out]
            n157 = Close Reference(reference=w461) -> ()  [unwired: 1 in, 1 out]
            n158 = invoke class="Pnl" method="Paste Selection"(reference=w468, error in=w469, "Pos"=T5 {"Left"=0, "Top"=0} ("Position")) -> (reference out=w465:refnum<vi>, error out=w464:errorcluster)  [unwired: 2 in, 3 out]
            n159 = property class="Pnl"(reference=w465, error in=w464) -> (reference out=w459:refnum<vi>, error out=w463:errorcluster, "Controls[]"=w467:refnum<vi>[])
            n160 = Index Array(array=w467) -> (element=w466:refnum<vi>)  [unwired: 1 in]
            n161 = property class="Ctl"(reference=w466, error in=w463, "Position"=w462) -> (reference out=w460:refnum<vi>, error out=w456:errorcluster)
            n162 = Close Reference(reference=w460, error in (no error)=w456) -> (error out=w485:errorcluster)
            n163 = Close Reference(reference=w459, error in (no error)=w485) -> (error out=w447:errorcluster)
            n164 = invoke class="VI" method="Save.Instrument"(reference=w446, error in=w447) -> (error out=w444:errorcluster)  [unwired: 4 in, 5 out]
            n165 = invoke class="LVClassLibrary" method="Save"(reference=w442, error in=w444) -> (error out=w443:errorcluster)  [unwired: 2 in, 3 out]
            n166 = Close Reference(reference=w446, error in (no error)=w443) -> (error out=w441:errorcluster)
            n167 = Close Reference(reference=w455, error in (no error)=w441) -> (error out=w457:errorcluster)
            n168 = Close Reference(reference=w454, error in (no error)=w457) -> (error out=w458:errorcluster)
            n169 = Close Reference(reference=w448, error in (no error)=w458) -> (error out=w440:errorcluster)
            n170 = invoke class="App" method="Clipboard.Empty"(error in=w440) -> ()  [unwired: 2 in, 3 out]
          }
          frame "UpdateIcons" {
            n171 = Unbundle By Name(w506) -> ("ClassRefnum"=w505:refnum<vi>)
            n172 = Unbundle By Name(w506) -> ("SubClass"=w510:bool, "ClassName"=w507:string)
            n173 = call-dynamic "ProgressWindow.vi"("ClassWriter in"=w493, "Message(Exit)"="Hide", "error in (no error)"=w497) -> ("ClassWriter out"=w499:refnum<class "ClassWriterNative.lvclass">, "error out"=w496:errorcluster)  [unwired: 15 in]
            n174 = Empty String/Path?(string/path=w502) -> (empty?=w503:bool)
            n175 = Not(x=w503) -> (.not. x?=w501:bool)
            n176 = call <resource>:"GDSLvIcon_DialogUpdateClass.vi"("ClassPath(FilePath/ProjectTreePath/LvCLassRef)"=w505, "ClassName"=w507, "AutoUpdate"=w501, "error in (no error)"=w496, "HeaderToApply (take from VIRef or /use 2D-8bit header, Ignored if not wired)"=w502) -> ("error out"=w495:errorcluster)  [unwired: 11 in, 3 out]
            n177 = Select(t="ReplaceBaseTemplateReferences", s=w510, f="AddFolders") -> (s? t:f=w508:string)
            n178 = call-dynamic "ProgressWindow.vi"("ClassWriter in"=w499, "Message(Exit)"="UnHide", "error in (no error)"=w495) -> ("error out"=w494:errorcluster)  [unwired: 15 in, 1 out]
          }
          frame "ReplaceBaseTemplateReferences" {
            # "This is a sub class, replace all BaseClass References with Select base class.\nIf base not equal to root, also replace BaseClass ObjectRef with Root-Base ObjectRef"
            n179 = Unbundle By Name(w525) -> ("VIs"=w530:refnum<vi>[], "TemplateClass"=w514:refnum<vi>, "BaseClassFolder"=w524:path, "BaseClassName"=w527:string)
            n180 = Unbundle By Name(w525) -> ()  [unwired: 1 out]
            n181 = property class="LVClassLibrary"(reference=w514) -> ("Parent"=w513:refnum<vi>)  [unwired: 1 in, 2 out]
            n182 = property class="LVClassLibrary"(reference=w513) -> (reference out=w511:refnum<vi>, error out=w512:errorcluster, "Name"=w517:string)  [unwired: 1 in]
            n183 = Format Into String(LvNativeTemplateNames."NativeBaseTemplate" ("TemplateNames")) -> ()  [unwired: 3 in, 2 out]
            n184 = Close Reference(reference=w511, error in (no error)=w512) -> ()  [unwired: 1 out]
            n185 = Match Pattern(string=w517, regular expression="\\2E[Ll][Vv][Cc][Ll][Aa][Ss][Ss]$") -> (before substring=w515:string)  [unwired: 1 in, 3 out]
            n186 = call-dynamic "GetTemplatePath.vi"("reference in"=w520, "ClassTemplateSubDirectory"=w515, "error in (no error)"=w518) -> ("FolderPathOut"=w526:path, "error out"=w519:errorcluster)  [unwired: 12 in, 3 out]
            n187 = call <resource>:"GOOP300_FindFilesToExchange.vi"("OldClassName(Prefix or suffix for some VIs)"=w515, "OldFolderPath"=w526, "NewFolderPath"=w524, "NewClassName(Prefix or suffix for some VIs)"=w527) -> ("OldFiles"=w522:path[], "NewFileArray"=w521:path[])  [unwired: 14 in]
            n188 = for {
              tunnel: w530 -> [w535] mode=indexing
              shift-right: [w533] -> w529
              shift-left: w519 -> [w534]
              tunnel: w522 -> [w532]
              tunnel: w521 -> [w531]
              n189 = call <resource>:"Scripting_ReplaceVisAndControls.vi"("ViRef"=w535, "OldVIsAndControls"=w532, "NewVIsAndControls"=w531, "error in (no error)"=w534) -> ("error out"=w533:errorcluster)  [unwired: 14 in, 1 out]
            }
          }
          frame "AddFolders" {
            n190 = Unbundle By Name(w546) -> ("ClassRefnum"=w545:refnum<vi>)
            n191 = call <resource>:"GDSProject_CreateFolder.vi"("Project Item To Create Folder Below(Use MyComputer if not wired)"=w545, "FolderName"="private", "error in (no error)"=w544, "CreateThePhysicalFolderIfPossible(False)"=TRUE ("CreateThePfysicalFolderIfPossible(False)")) -> ("ItemOut"=w551:refnum<vi>, "error out"=w549:errorcluster)  [unwired: 12 in, 2 out]
            n192 = invoke class="LVClassLibrary" method="Set Source Scope"(reference=w545, error in=w549, "SourceRef"=w551, "Scope"=T4."private" ("scope")) -> (reference out=w536:refnum<vi>, error out=w539:errorcluster)  [unwired: 1 in, 3 out]
            n193 = call <resource>:"GDSProject_CreateFolder.vi"("Project Item To Create Folder Below(Use MyComputer if not wired)"=w536, "FolderName"="protected", "error in (no error)"=w539, "CreateThePhysicalFolderIfPossible(False)"=TRUE ("CreateThePfysicalFolderIfPossible(False)")) -> ("ItemOut"=w541:refnum<vi>, "error out"=w542:errorcluster)  [unwired: 12 in, 2 out]
            n194 = invoke class="LVClassLibrary" method="Set Source Scope"(reference=w536, error in=w542, "SourceRef"=w541, "Scope"=T4."protected" ("scope")) -> (error out=w538:errorcluster)  [unwired: 1 in, 4 out]
          }
          frame "SetClassProperties" {
            n195 = Unbundle By Name(w580) -> ("ClassDescription"=w576:string, "ParentInterfaces"=w553:path[])
            n196 = Unbundle By Name(w560) -> ("ClassRefnum"=w567:refnum<vi>)
            n197 = Unbundle By Name(w560) -> ("TemplateName"=w575:string, "SubClass"=w585:bool)
            n198 = Unbundle By Name(w560) -> ("BaseClassFolder"=w584:path)
            n199 = Unbundle By Name(w560) -> ("TemplateClass"=w574:refnum<vi>)
            n200 = property class="LVClassLibrary"(reference=w574) -> ("Version"=w573:T11)  [unwired: 1 in, 2 out]
            n201 = case shown="False" w585 {
              tunnel: w567 -> [w592 w602]
              tunnel: [w592 w601] -> w582
              tunnel: w566 -> [w589 w599]
              tunnel: [w588 w598] -> w581
              tunnel: w584 -> [_ w600]
              tunnel: [w587 w594] -> w561
              frame False {
                n202 = call <resource>:"BaseProvider_ConfigurationMemory.vi"("error in (no error)"=w589, "Action"=enum16{"Read", "Load", "Save"}."Read") -> ("PatternOut"=w591:T12, "error out"=w588:errorcluster)  [unwired: 11 in, 5 out]
                n203 = Format Into String(w591) -> (resulting string=w587:string)  [unwired: 3 in, 1 out]
              }
              frame True {
                n204 = call <resource>:"GDSProject_OpenClass.vi"("ClassPath(FilePath/ProjectTreePath/LvCLassRef)"=w600, "error IO"=w599) -> ("LVClass.Open"=w597:refnum<vi>, "error out"=w596:errorcluster)  [unwired: 15 in, 1 out]
                n205 = call <resource>:"GDSLvClass_ReadClassType.vi"("Class Refnum In"=w597) -> ("Class Refnum Out"=w595:refnum<vi>, "ClassSettings"=w593:T7)  [unwired: 16 in, 1 out]
                n206 = property class="LVClassLibrary"(reference=w602, error in=w596, "Parent"=w595) -> (reference out=w601:refnum<vi>, error out=w598:errorcluster)
                n207 = Unbundle By Name(w593) -> ("ConnectorPanePattern"=w594:string)
                n208 = Close Reference(reference=w595, error in (no error)=w598) -> ()  [unwired: 1 out]
              }
            }
            n209 = Unbundle(w573) -> ("Major"=w571:u16, "Minor"=w570:u16, "Fix"=w569:u16, "Build"=w568:u16)
            n210 = Format Into String(format string="%d.%d.%d.%d", w571, w570, w569, w568) -> (resulting string=w558:string)  [unwired: 2 in, 1 out]
            n211 = Format Into String(LvNativeProviderName."Endevo LabVIEW Native" ("ProviderName")) -> (resulting string=w577:string)  [unwired: 3 in, 1 out]
            n212 = Bundle By Name(cluster=T7 {"ClassProviderName"="", "ClassTemplateUsed"="", "ClassTemplateVersion"="", "ClassDescription"="", "PlugIns"=[], "ConnectorPanePattern"=""} ("ClassSettings"), "ClassProviderName"=w577, "ClassTemplateUsed"=w575, "ClassTemplateVersion"=w558, "ClassDescription"=w576, "ConnectorPanePattern"=w561) -> (w578:T7)
            n213 = Bundle By Name(cluster=w560, "TemplateVersionUsed"=w558) -> (w559:T2)
            n214 = call <resource>:"GDSLvClass_StoreClassType.vi"("Class Refnum In"=w582, "ClassSettings"=w578, "CheckAndFixConnectorPaneType(False)"=TRUE, "error in (no error)"=w581) -> ("Class Refnum Out"=w564:refnum<vi>, "error out"=w563:errorcluster)  [unwired: 14 in]
            n215 = call <resource>:"UpdateClassApperance.vi"("ClassRefIn"=w564, "error in (no error)"=w563) -> ("ClassRefOut"=w555:refnum<vi>, "error out"=w562:errorcluster)  [unwired: 16 in]
            n216 = call <resource>:"SetParentInterfaces.vi"("error in"=w562, "Parent Interfaces(ClassRef/Path)"=w553, "Class/InterfaceRefIn"=w555) -> ("error out"=w556:errorcluster, "Class/InterfaceRefOut"=w554:refnum<vi>)  [unwired: 7 in]
            n217 = invoke class="LVClassLibrary" method="Save"(reference=w554, error in=w556) -> (error out=w583:errorcluster)  [unwired: 2 in, 3 out]
          }
          frame "FixAttribute" {
            w631 = refnum<vi> refnum  # Control
            w635 = refnum<vi> refnum  # Cluster
            # "JUST BECASUSE IT FAILS SOMETIMES"
            n218 = Unbundle By Name(w637) -> ("ClassRefnum"=w614:refnum<vi>)
            n219 = property class="LVClassLibrary"(reference=w614, error in=w615) -> (error out=w643:errorcluster, "Member Data"=w606:refnum<vi>)  [unwired: 1 out]
            n220 = property class="VI"(reference=w606, error in=w643, "Front Panel.Open"=FALSE ("Front Panel Window:Open")) -> (error out=w611:errorcluster, "Panel"=w641:refnum<vi>)  [unwired: 1 out]
            n221 = property class="Pnl"(reference=w641, error in=w611) -> (reference out=w619:refnum<vi>, error out=w626:errorcluster, "Controls[]"=w642:refnum<vi>[])
            n222 = Index Array(array=w642) -> (element=w636:refnum<vi>)  [unwired: 1 in]
            n223 = To More Specific Class(target class=w635, reference=w636, error in=w626) -> (specific class reference=w634:refnum<vi>, error out=w627:errorcluster)
            n224 = property class="Clust"(reference=w634, error in=w627) -> (reference out=w621:refnum<vi>, error out=w628:errorcluster, "AllObjs[]"=w633:refnum<vi>[])
            n225 = Index Array(array=w633) -> (element=w632:refnum<vi>)  [unwired: 1 in]
            n226 = To More Specific Class(target class=w631, reference=w632, error in=w628) -> (specific class reference=w630:refnum<vi>, error out=w629:errorcluster)
            n227 = property class="Ctl"(reference=w630, error in=w629) -> (reference out=w625:refnum<vi>, error out=w624:errorcluster, "Label.Text"=w623:string, "Label.Left"=w604:i32)
            n228 = disable-structure shown="Enabled" {
              disable-tunnel: w625 -> [w651 w652]
              disable-tunnel: w624 -> [w649 w653]
              disable-tunnel: [w648 w652] -> w613
              disable-tunnel: [w646 w653] -> w612
              disable-tunnel: w606 -> [w645 _]
              frame Disabled {
                n229 = property class="Ctl"(reference=w651, error in=w649, "Label.Text"="UpdateMe") -> (reference out=w648:refnum<vi>, error out=w647:errorcluster)
                n230 = invoke class="VI" method="Save.Instrument"(reference=w645, error in=w647) -> (error out=w646:errorcluster)  [unwired: 4 in, 5 out]
              }
              frame Enabled {
              }
            }
            n231 = Increment(x=w604) -> (x+1=w603:i32)
            n232 = property class="Ctl"(reference=w613, error in=w612, "Label.Text"=w623, "Label.Left"=w603) -> (reference out=w608:refnum<vi>, error out=w622:errorcluster)
            n233 = Close Reference(reference=w608, error in (no error)=w622) -> (error out=w607:errorcluster)
            n234 = invoke class="VI" method="Save.Instrument"(reference=w606, error in=w607) -> (error out=w605:errorcluster)  [unwired: 4 in, 5 out]
            n235 = invoke class="VI" method="CtlVIApplyChanges"(reference=w606, error in=w605) -> (reference out=w610:refnum<vi>, error out=w609:errorcluster)  [unwired: 1 in, 1 out]
            n236 = Close Reference(reference=w621, error in (no error)=w609) -> (error out=w620:errorcluster)
            n237 = Close Reference(reference=w619, error in (no error)=w620) -> (error out=w618:errorcluster)
            n238 = invoke class="VI" method="Save.Instrument"(reference=w610, error in=w618) -> (reference out=w617:refnum<vi>, error out=w639:errorcluster)  [unwired: 4 in, 4 out]
            n239 = invoke class="LVClassLibrary" method="Save"(reference=w614, error in=w639) -> (error out=w638:errorcluster)  [unwired: 2 in, 3 out]
            n240 = Close Reference(reference=w617, error in (no error)=w638) -> (error out=w616:errorcluster)
          }
          frame "CloseRefs", "Error", Default {
            n241 = case shown="Default" w662 {
              tunnel: w668 -> [w676 w683]
              tunnel: w659 -> [w675 w684]
              tunnel: [w674 w683] -> w658
              frame "CloseRefs" {
                n242 = Unbundle By Name(w675) -> ("VIs"=w677:refnum<vi>[])
                n243 = for {
                  tunnel: w677 -> [w680] mode=indexing
                  shift-right: [w682] -> w674
                  shift-left: w676 -> [w681]
                  n244 = invoke class="VI" method="Save.Instrument"(reference=w680, error in=w681) -> (reference out=w678:refnum<vi>, error out=w679:errorcluster)  [unwired: 4 in, 4 out]
                  n245 = Close Reference(reference=w678, error in (no error)=w679) -> (error out=w682:errorcluster)
                }
              }
              frame Default {
                n246 = Unbundle By Name(w684) -> ("VIs"=w685:refnum<vi>[])
                n247 = for {
                  tunnel: w685 -> [w686] mode=indexing
                  n248 = Close Reference(reference=w686) -> ()  [unwired: 1 in, 1 out]
                }
              }
            }
            n249 = Unbundle By Name(w659) -> ("App"=w654:refnum<vi>, "TemplateClass"=w667:refnum<vi>, "ProjectRefnum"=w664:refnum<vi>, "ClassRefnum"=w663:refnum<vi>)
            n250 = case shown="True" w657 {
              tunnel: [w672 w673] -> w666
              tunnel: w663 -> [w671 _]
              tunnel: w658 -> [w670 w673]
              frame False {
                n251 = Close Reference(reference=w671, error in (no error)=w670) -> (error out=w672:errorcluster)
              }
              frame True {
              }
            }
            n252 = Close Reference(reference=w664, error in (no error)=w666) -> (error out=w665:errorcluster)
            n253 = Close Reference(reference=w667, error in (no error)=w665) -> (error out=w656:errorcluster)
            n254 = Close Reference(reference=w654, error in (no error)=w656) -> (error out=w655:errorcluster)
            n255 = call <resource>:"GDSError_LogErrorInformation.vi"("State"=w660, "LocalVariableData"=w659, "error in (no error)"=w655) -> ("error out"=w661:errorcluster)  [unwired: 16 in]
          }
        }
        n256 = Equal?(x=w31, y="Exit") -> (x = y?=w35:bool)
        n257 = Select(t="Error", s=w30, f=w31) -> (s? t:f=w34:string)
      }
    }
    frame Error {
    }
  }
  "error out" <- w7
  n258 = Unbundle By Name(w3) -> ("ClassRefnum"=→"LVClassLibraryRefnum":refnum<vi>, "TemplateVersionUsed"=→"TemplateVersionUsed":string)
  "ClassWriterNative" <- "ClassWriterNative"
